vi "Clean Project.vi"(8 "error in":errorcluster, 11 "Runner in":refnum<class "Runner.lvclass">) -> (0 "error out":errorcluster, 3 "Runner out":refnum<class "Runner.lvclass">)   [LabVIEW 2026, in "Runner.lvlib" / "Runner.lvclass"]
doc: "Remove template files from project folder."
uses:
  Runner.lvclass
  Runner.lvclass/Runner.ctl
  Interfaces/ILogger/ILogger Messages/Log Msg/Log Msg.lvclass/Log Msg.ctl
  <vilib>/ActorFramework/Message Enqueuer/Message Enqueuer.lvclass/Message Enqueuer.ctl
  <vilib>/ActorFramework/Message Enqueuer/Enqueue.vi
  Interfaces/ILogger/ILogger Messages/Log Msg/Log Msg.lvclass
  <vilib>/ActorFramework/Message Priority Queue/Priority Enqueue.vi
  Interfaces/IFile Manager/IFile Manager.lvclass
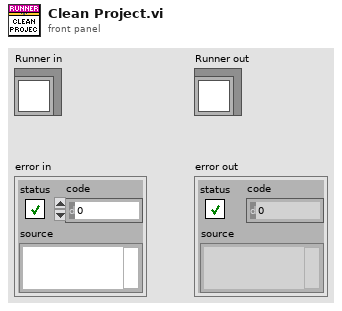
[diagram p1: front panel]
types:
  T1 = typedef "Log Entry--cluster.ctl" = cluster{"Time":timestamp, "Message":string}
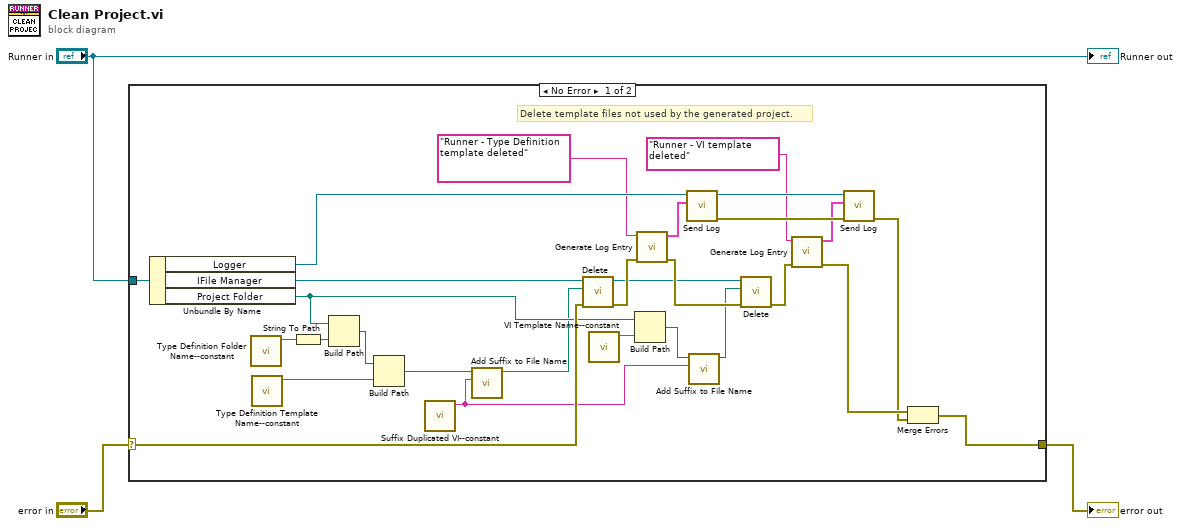
[diagram p0: block diagram]
diagram:
  n1 = case shown="No Error" "error in" {
    selector: "error in" -> [w24 w32]
    tunnel: [w29 w32] -> w3
    tunnel: "Runner in" -> [w23 _]
    frame No Error {
      # "Delete template files not used by the generated project."
      n2 = Unbundle By Name(w23) -> ("Logger"=w20:refnum<class "Message Enqueuer.lvclass">, "IFile Manager"=w10:refnum<class "IFile Manager.lvclass">, "Project Folder"=w12:path)
      n3 = call "Type Definition Folder Name--constant.vi"() -> ("Type Definition Folder Name"=w22:string)  [unwired: 11 in]
      n4 = call "Type Definition Template Name--constant.vi"() -> ("Type Definition Template Name"=w21:string)  [unwired: 11 in]
      n5 = String To Path(string=w22) -> (path=w14:path)
      n6 = Build Path(base path=w12, name or relative path=w14) -> (appended path=w13:path)
      n7 = Build Path(base path=w13, name or relative path=w21) -> (appended path=w8:path)
      n8 = call "Suffix Duplicated VI--constant.vi"() -> ("Suffix Duplicated VI"=w4:string)  [unwired: 11 in]
      n9 = call "Add Suffix to File Name.vi"("Suffix"=w4, "File Path in"=w8) -> ("File Path out"=w7:path)  [unwired: 9 in]
      n10 = call-dynamic "Delete.vi"("error in"=w24, "Path"=w7, "IFile Manager in"=w10) -> ("error out"=w27:errorcluster, "IFile Manager out"=w9:refnum<class "IFile Manager.lvclass">)  [unwired: 7 in]
      n11 = call "VI Template Name--constant.vi"() -> ("VI Template Name"=w11:string)  [unwired: 11 in]
      n12 = Build Path(base path=w12, name or relative path=w11) -> (appended path=w6:path)
      n13 = call "Generate Log Entry.vi"("error in"=w27, "Message"="Runner - Type Definition template deleted") -> ("error out"=w26:errorcluster, "Log Entry"=w17:T1)  [unwired: 8 in]
      n14 = call "Send Log.vi"("Log Entry"=w17, "Message Enqueuer"=w20) -> ("error out"=w31:errorcluster, "Message Enqueuer out"=w19:refnum<class "Message Enqueuer.lvclass">)  [unwired: 8 in]
      n15 = call "Add Suffix to File Name.vi"("Suffix"=w4, "File Path in"=w6) -> ("File Path out"=w5:path)  [unwired: 9 in]
      n16 = call-dynamic "Delete.vi"("error in"=w26, "Path"=w5, "IFile Manager in"=w9) -> ("error out"=w25:errorcluster)  [unwired: 7 in, 1 out]
      n17 = call "Generate Log Entry.vi"("error in"=w25, "Message"="Runner - VI template deleted") -> ("error out"=w30:errorcluster, "Log Entry"=w15:T1)  [unwired: 8 in]
      n18 = call "Send Log.vi"("error in (no error)"=w31, "Log Entry"=w15, "Message Enqueuer"=w19) -> ("error out"=w28:errorcluster)  [unwired: 7 in, 1 out]
      n19 = Merge Errors(w30, w28) -> (w29:errorcluster)
    }
    frame Error {
      # "Pass error without further actions."
    }
  }
  "error out" <- w3
  "Runner out" <- "Runner in"
